vi "Performance Values.vi"(8 "error in (no error)":errorcluster, 11 "Windows System SAL in":refnum<class "Windows System SAL.lvclass">) -> (0 "error out":errorcluster, 2 "Performance Values":T1)   [LabVIEW 2020, in "Volatus.lvlib" / "Windows System SAL.lvclass"]
uses:
  Windows System SAL.lvclass
  System SAL/Performance Values.ctl
  Windows System SAL.lvclass/Windows System SAL.ctl
  <vilib>/Analysis/baseanly.llb/Mean (DBL).vi
  System SAL/System SAL.lvclass
  <resource>/objmgr/nisysapi.rc
  <vilib>/Analysis/NI_AALBase.lvlib
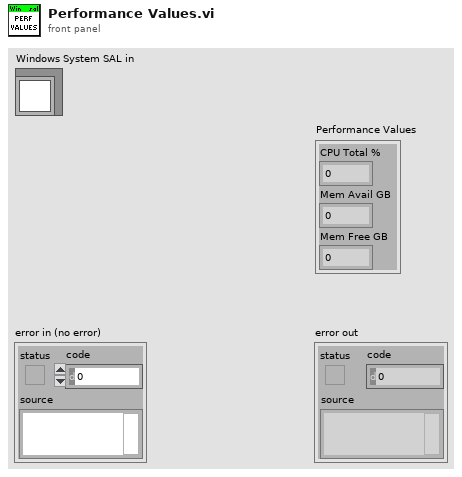
[diagram p1: front panel]
types:
  T1 = typedef "Volatus.lvlib/System SAL.lvclass/Performance Values.ctl" = cluster{"CPU Total %":dbl, "Mem Avail GB":dbl, "Mem Free GB":dbl}
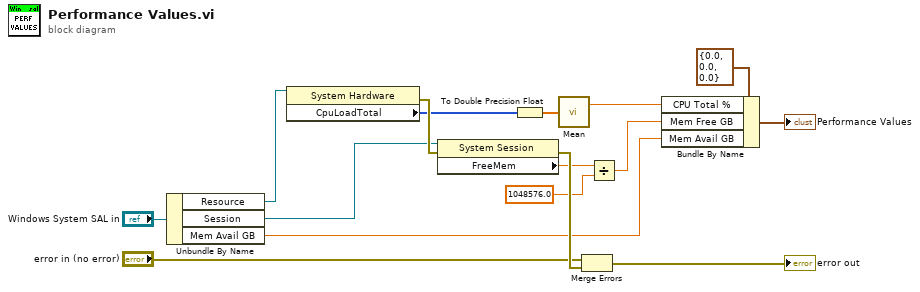
[diagram p0: block diagram]
diagram:
  n1 = Unbundle By Name("Windows System SAL in") -> ("Resource"=w10:refnum<k20>, "Session"=w6:refnum<k21>, "Mem Avail GB"=w5:dbl)
  n2 = property class="System Hardware"(reference=w10) -> (error out=w15:errorcluster, "CpuLoadTotal"=w9:u32[])  [unwired: 1 in, 1 out]
  n3 = property class="System Session"(reference=w6, error in=w15) -> (error out=w16:errorcluster, "FreeMem"=w3:dbl)  [unwired: 1 out]
  n4 = To Double Precision Float(number=w9) -> (double precision float=w8:dbl[])
  n5 = call-poly <vilib>:"Mean.vi"("X"=w8) -> ("mean"=w7:dbl)  [unwired: 1 out]
  n6 = Merge Errors("error in (no error)", w16) -> (→"error out":errorcluster)
  n7 = Divide(x=w3, y=1048576.0) -> (x/y=w1:dbl)
  n8 = Bundle By Name(cluster=T1 {"CPU Total %"=0.0, "Mem Avail GB"=0.0, "Mem Free GB"=0.0} ("Performance Values"), "CPU Total %"=w7, "Mem Free GB"=w1, "Mem Avail GB"=w5) -> (→"Performance Values":T1)
